vi "Digital_Read.vi"(8 "error in (no error)":errorcluster, 10 "Canal":u8, 11 "VISA resource name":refnum<visa-resource-name>) -> (0 "error out":errorcluster, 2 "Out":bool, 3 "VISA resource name out":refnum<visa-resource-name>)   [LabVIEW 2026]
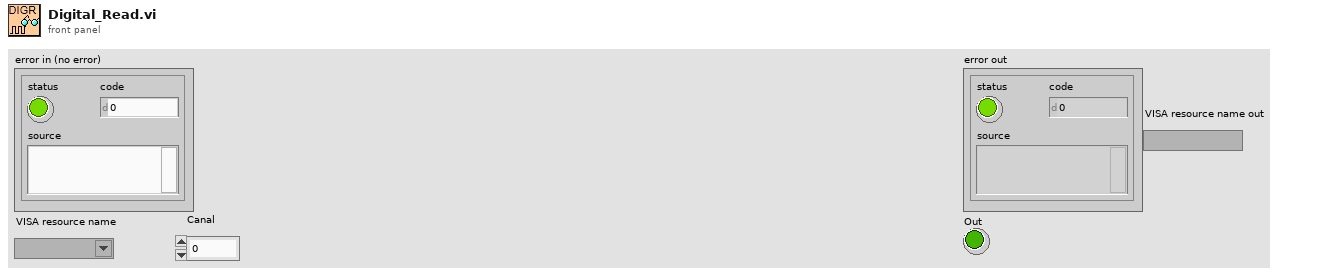
[diagram p1: front panel]
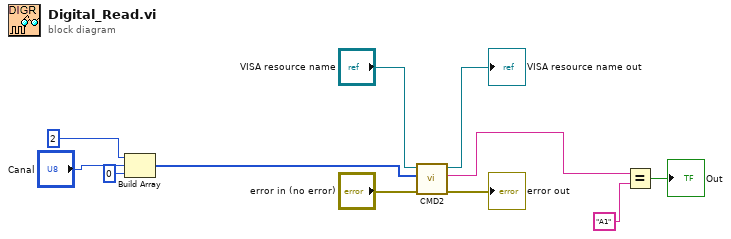
[diagram p0: block diagram]
diagram:
  n1 = Build Array(u8 2, "Canal", u8 0 ("element")) -> (w2:u8[])
  n2 = call "CMD2.vi"("error in (no error)"="error in (no error)", "Comando"=w2, "VISA resource name"="VISA resource name") -> ("error out"=→"error out":errorcluster, "respuesta"=w7:string, "VISA resource name out"=→"VISA resource name out":refnum<visa-resource-name>)  [unwired: 6 in]
  n3 = Equal?(x=w7, y="A1") -> (x = y?=→"Out":bool)
